vi "Free File Path Str.vi"(8 "error in (no error)":errorcluster caption="错误输入（无错误）", 11 "strFilePath":string) -> (0 "error out":errorcluster caption="错误输出", 3 "strFilePath out":string)   [LabVIEW 2017, in "smncsftmt.lvlib"]
doc: "__declspec(dllexport) void FreeFilePathStr(char* strFilePath);"
uses:
  smncsftmt.lvlib
  smncsftmt.dll
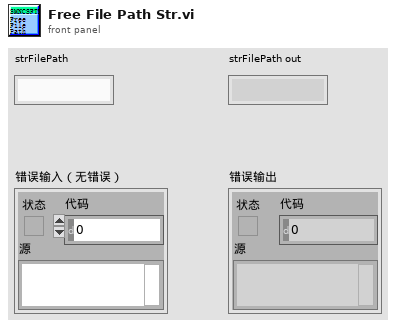
[diagram p1: front panel]
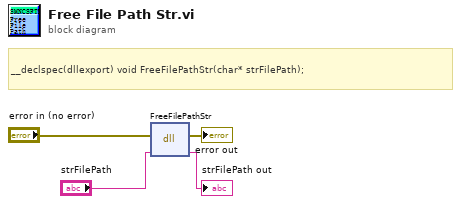
[diagram p0: block diagram]
diagram:
  # "__declspec(dllexport) void FreeFilePathStr(char* strFilePath);"
  n1 = dll-call lib="PTH2oabs CUsersaDesktop\nLABVIEW范例National InstrumentsLabVIEW 2017user.lib\tsmncsftmtsmncsftmt.*" fn="FreeFilePathStr"(error in="error in (no error)", "strFilePath"="strFilePath") -> (error out=→"error out":errorcluster, "strFilePath"=→"strFilePath out":string)  [unwired: 3 in, 1 out]
